vi "lvmcp_sradd.vi"() -> ()   [LabVIEW 2026]
panel:
  out "error out":errorcluster
  in  "reference":refnum<vi>
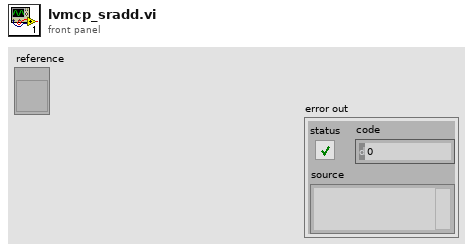
[diagram p1: front panel]
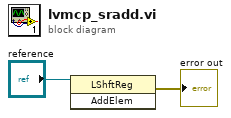
[diagram p0: block diagram]
diagram:
  n1 = invoke class="LShftReg" method="AddElem"(reference="reference") -> (error out=→"error out":errorcluster)  [unwired: 2 in, 2 out]
